vi "俄罗斯方块-存储形状数组.vi"(6 "Y":i8, 7 "X":i8, 8 "当前形状数组":u32[][](array[numeric]), 9 "主窗数组输入":u32[][](array[colorbox])) -> (0 "是否溢出":bool, 3 "主窗数组输出":u32[][](array[colorbox]))   [LabVIEW 2021]
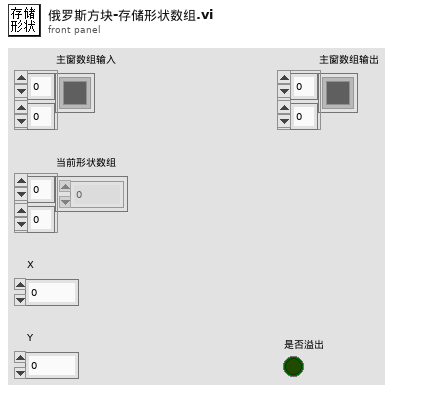
[diagram p1: front panel]
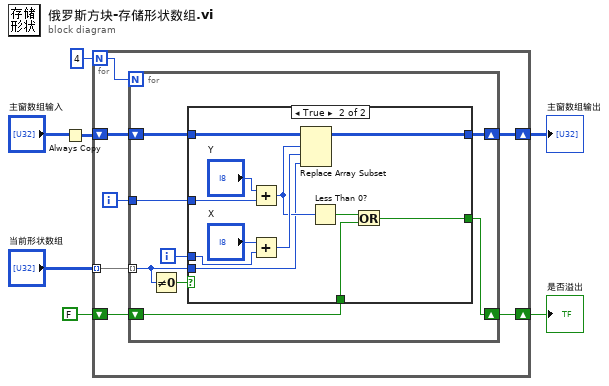
[diagram p0: block diagram]
diagram:
  n1 = Always Copy(1:"主窗数组输入") -> (0:w5:u32[][])
  n2 = for {
    N: 4 -> [w14]
    tunnel: "当前形状数组" -> [w13] mode=indexing
    shift-right: [w11] -> w7
    shift-left: w5 -> [w12]
    shift-right: [w8] -> w2
    shift-left: FALSE -> [w9]
    i -> [w10]
    n3 = for {
      N: w14 -> [_]
      tunnel: w13 -> [w20] mode=indexing
      shift-right: [w19] -> w11
      shift-left: w12 -> [w21]
      tunnel: w10 -> [w18]
      shift-right: [w15] -> w8
      shift-left: w9 -> [w16]
      i -> [w17]
      n4 = Not Equal To 0?(x=w20) -> (x != 0?=w22:bool)
      n5 = case shown="True" w22 {
        tunnel: w21 -> [w24 w36]
        tunnel: w20 -> [_ w27]
        tunnel: [w24 w35] -> w19
        tunnel: w18 -> [_ w34]
        tunnel: w17 -> [_ w33]
        tunnel: w16 -> [w23 w26]
        tunnel: [w23 w25] -> w15
        frame False {
        }
        frame True {
          n6 = Add(x="Y", y=w34) -> (x+y=w29:i32)
          n7 = Add(x="X", y=w33) -> (x+y=w32:i32)
          n8 = Replace Array Subset(array=w36, new element=w27, index (row)=w29, index (col)=w32) -> (w35:u32[][])
          n9 = Less Than 0?(x=w29) -> (x < 0?=w28:bool)
          n10 = Or(x=w28, y=w26) -> (x .or. y?=w25:bool)
        }
      }
    }
  }
  "主窗数组输出" <- w7
  "是否溢出" <- w2
